vi "ADB List Device.vi"(11 "ADB Path":string="C:\\Projects\\Maestro\\PLTS\\ADB\\support") -> (3 "ADB Devices":T1(array[cluster]))   [LabVIEW 2018]
uses:
  <vilib>/regexp/Match Regular Expression.xnode
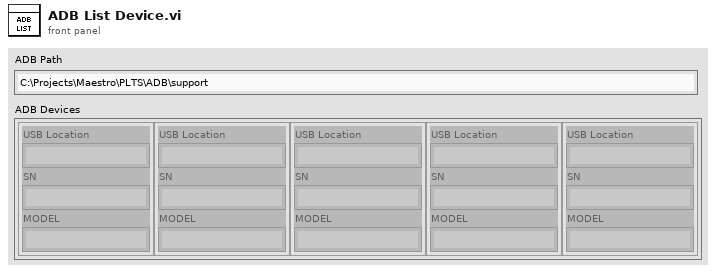
[diagram p1: front panel]
types:
  T1 = cluster{"USB Location":string, "SN":string, "MODEL":string}[]
  T2 = cluster{"USB Location":string, "SN":string, "MODEL":string}
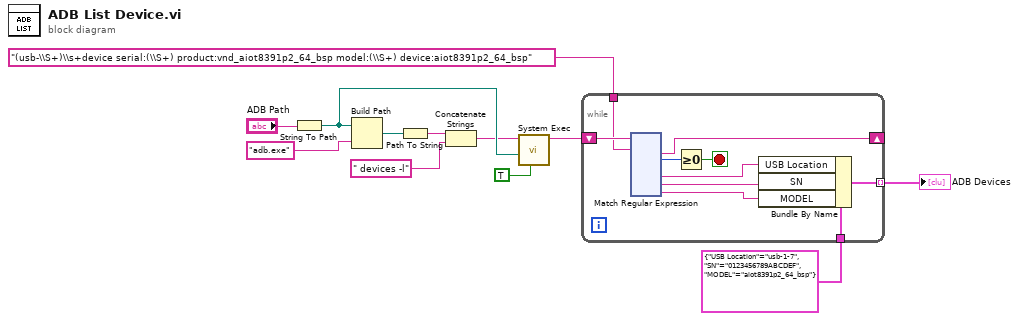
[diagram p0: block diagram]
diagram:
  n1 = String To Path(string="ADB Path") -> (path=w10:path)
  n2 = Build Path(base path=w10, name or relative path="adb.exe") -> (appended path=w9:path)
  n3 = Path To String(path=w9) -> (string=w8:string)
  n4 = Concatenate Strings(w8, " devices -l") -> (w6:string)
  n5 = call <vilib>:"System Exec.vi"("run minimized? (F)"=TRUE, "working directory"=w10, "command line"=w6) -> ("standard output"=w4:string)  [unwired: 5 in, 3 out]
  n6 = while {
    tunnel: "(usb-\\S+)\\s+device serial:(\\S+) product:vnd_aiot8391p2_64_bsp model:(\\S+) device:aiot8391p2_64_bsp" -> [w21]
    shift-right: [w20] -> _
    shift-left: w4 -> [w22]
    tunnel: [w14] -> w1 mode=indexing
    tunnel: T2 {"USB Location"="usb-1-7", "SN"="0123456789ABCDEF", "MODEL"="aiot8391p2_64_bsp"} ("ADB Device") -> [w13]
    stop <- w18 stop-if-true
    n7 = xnode "Match Regular Expression"("input string"=w22, "regular expression"=w21) -> ("after match"=w20:string, "offset past match"=w19:i32, "submatch 1"=w17:string, "submatch 2"=w16:string, "submatch 3"=w15:string)  [unwired: 4 in, 3 out]
    n8 = Greater Or Equal To 0?(x=w19) -> (x >= 0?=w18:bool)
    n9 = Bundle By Name(cluster=w13, "USB Location"=w17, "SN"=w16, "MODEL"=w15) -> (w14:T2)
  }
  "ADB Devices" <- w1
